vi "GMAP_API_Dispose_MapRef (SubVI).vi"(8 "error in":errorcluster, 11 "map file path":path) -> (0 "error out":errorcluster)   [LabVIEW 2025]
doc: "This VI deletes HTML file, containing Google map,\ncreated by the GMAP_API_CreateMapRef (SubVI)"
panel:
  # "This VI deletes HTML file, containing Google map,\ncreated by the GMAP_API_CreateMapRef (SubVI)"
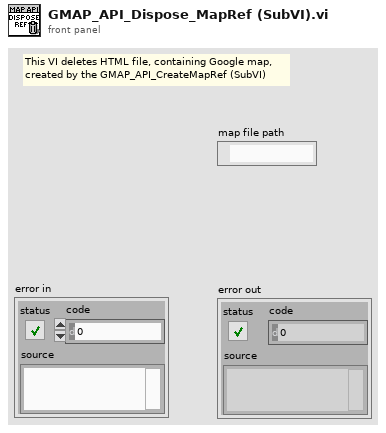
[diagram p1: front panel]
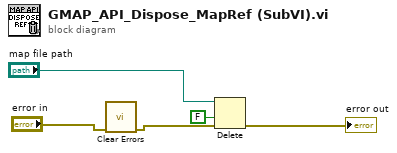
[diagram p0: block diagram]
diagram:
  n1 = call <vilib>:"Clear Errors.vi"("error in (no error)"="error in") -> ("error out"=w1:errorcluster)  [unwired: 5 in, 1 out]
  n2 = Delete(path (use dialog)="map file path", confirm (F)=FALSE, error in=w1) -> (error out=→"error out":errorcluster)  [unwired: 2 in, 2 out]
